vi "EJERCICIO _3_CREACION_VISUALIZACION_ARREGLO.vi"() -> ()   [LabVIEW 2026]
panel:
  out "ARREGLO INDICADOR":dbl[](array[numeric])
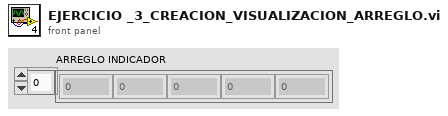
[diagram p1: front panel]
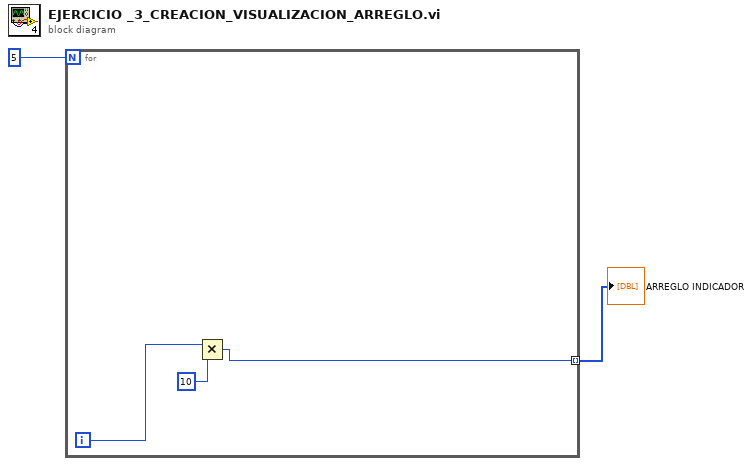
[diagram p0: block diagram]
diagram:
  n1 = for {
    N: 5 -> [_]
    tunnel: [w3] -> w1 mode=indexing
    i -> [w5]
    n2 = Multiply(x=w5, y=10) -> (x*y=w3:i32)
  }
  "ARREGLO INDICADOR" <- w1
